vi "SeqEditor_StepOpen.vi"(8 "error in (no error)":errorcluster, 11 "NLTest in":refnum<class "NLTest.lvclass">) -> (0 "error out":errorcluster, 3 "NLTest out":refnum<class "NLTest.lvclass">)   [LabVIEW 2017, in "NLTest.lvclass"]
uses:
  NLTest.lvclass
  NLTest.lvclass/NLTest.ctl
  VISTEP.ctl
  VISTEP_class_INOUTPUT.ctl
  VISTEP_class_INOUTPUT_TYPE.ctl
  VISTEP_class_steptestclass.ctl
panel:
  # "某个步骤被打开，加载PARAM MLST"
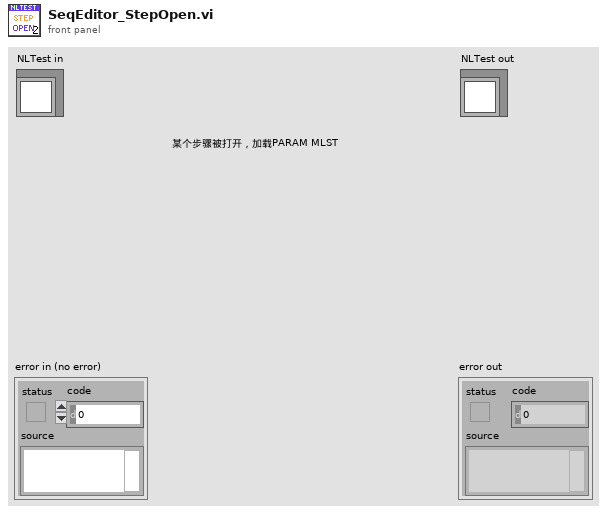
[diagram p1: front panel]
types:
  T1 = typedef "NLTest.lvclass/VISTEP.ctl" = cluster{"My":cluster{"VIpath":T2, "VIname":T2, "Loop":T2, "Skip":T2, "FailStop":T2, "StepClass":T2, "StringTest-Source":T2, "StringTest-Lim":T2, "BoolTest-Source":T2, "BoolTest-Lim":T2, "NumberTest-OP":T2, "NumberTest-Source":T2, "NumberTest-LimA":T2, "NumberTest-LimB":T2}, "INPUT":T2[], "OUTPUT":T2[]}
  T2 = typedef "NLTest.lvclass/VISTEP_class_INOUTPUT.ctl" = cluster{"ITEM":string, "DATA":string, "TYPE":T3, "TYPEDATA":string, "SV":bool, "clusterchain":refnum<vi>[]}
  T3 = typedef "NLTest.lvclass/VISTEP_class_INOUTPUT_TYPE.ctl" = enum16{"Number", "String", "Bool", "Enum", "Path", "VISA", "NA"}
  T4 = typedef "NLTest.lvclass/VISTEP_class_steptestclass.ctl" = enum16{"NotaTest", "StringTest", "BoolTest", "NumberTest", "NULL"}
  T5 = cluster{"ITEM":string, "TYPE":T3, "TYPEDATA":string}
  T6 = cluster{"VIpath":T2, "VIname":T2, "Loop":T2, "Skip":T2, "FailStop":T2, "StepClass":T2, "StringTest-Source":T2, "StringTest-Lim":T2, "BoolTest-Source":T2, "BoolTest-Lim":T2, "NumberTest-OP":T2, "NumberTest-Source":T2, "NumberTest-LimA":T2, "NumberTest-LimB":T2}
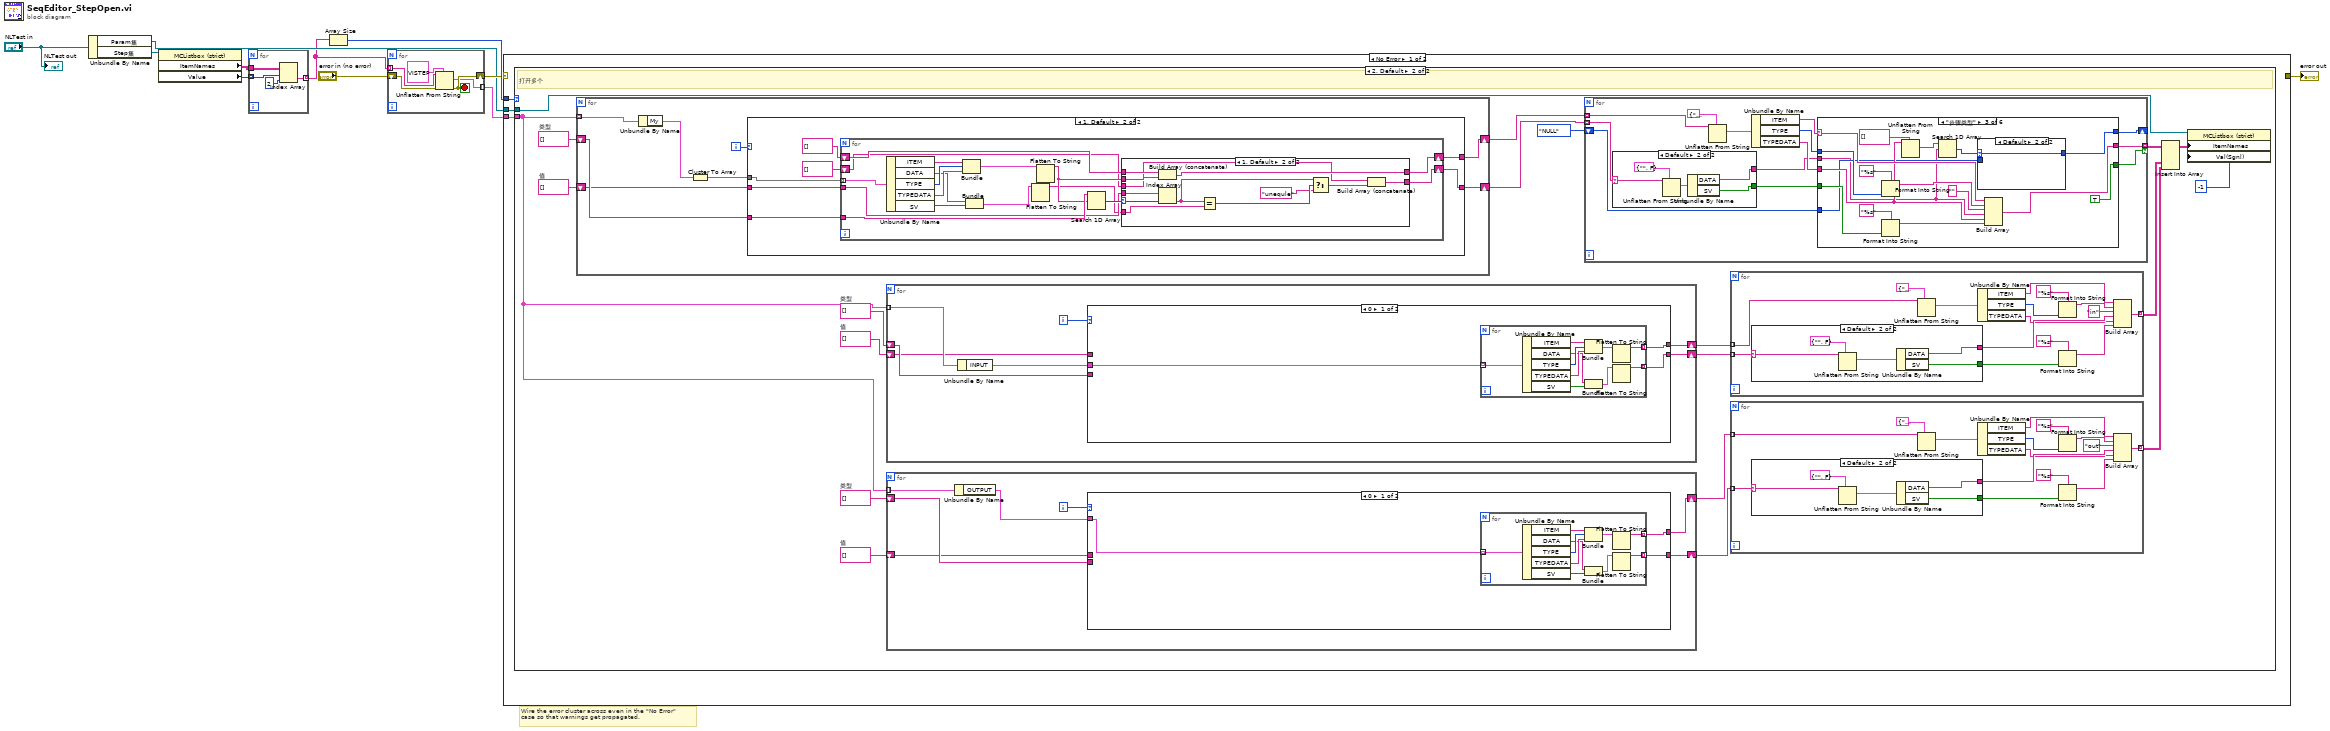
[diagram p0: block diagram]
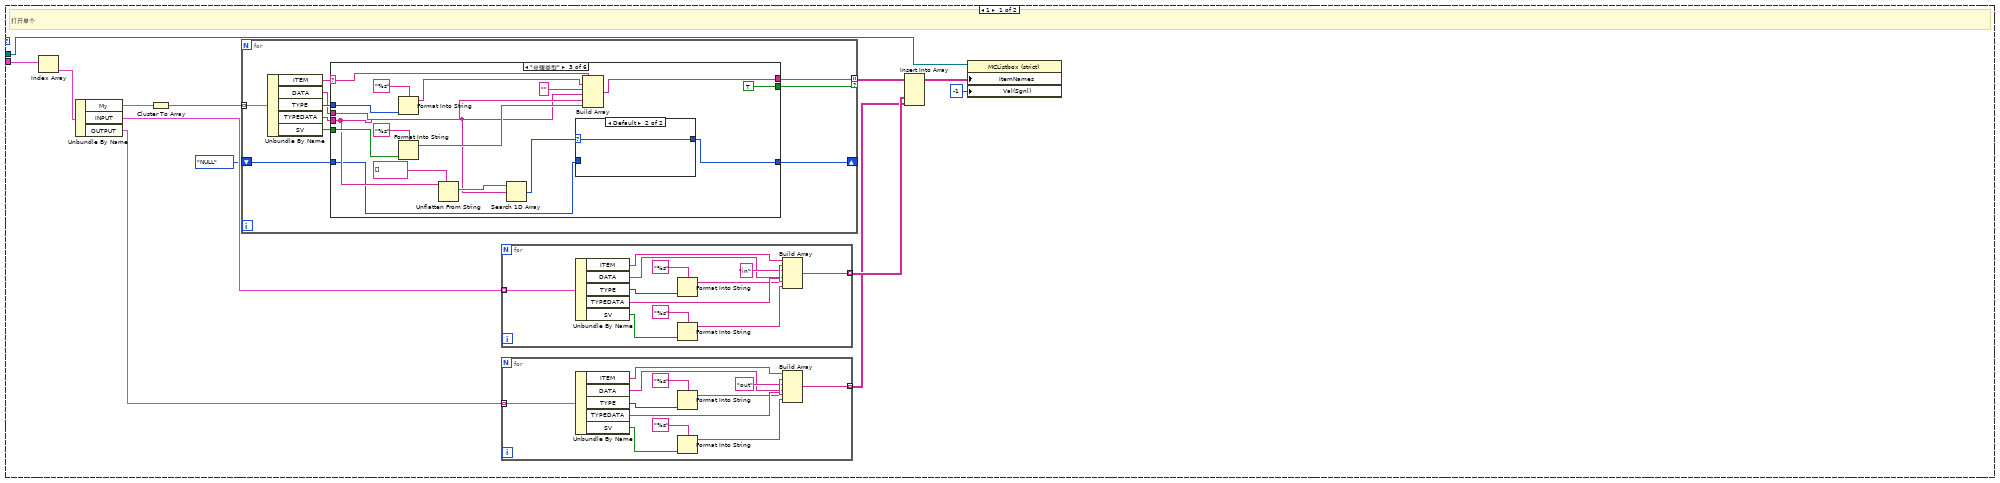
[diagram p2: hidden frame]
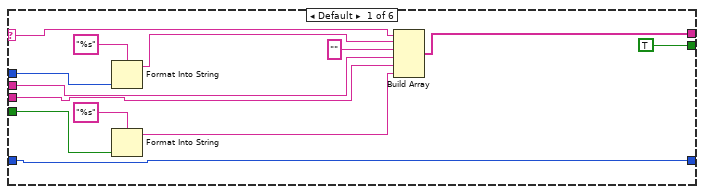
[diagram p3: hidden frame]
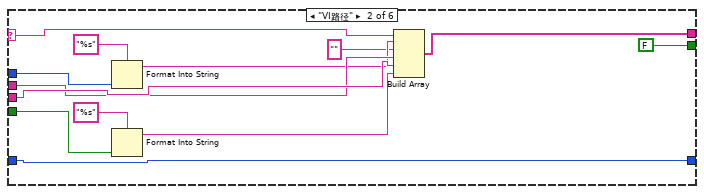
[diagram p4: hidden frame]
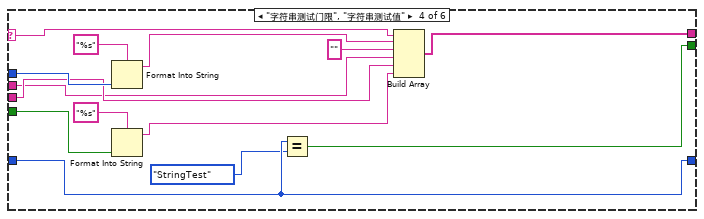
[diagram p6: hidden frame]
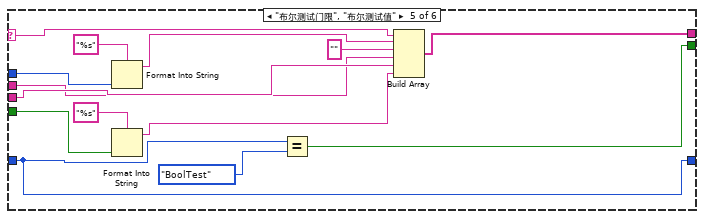
[diagram p7: hidden frame]
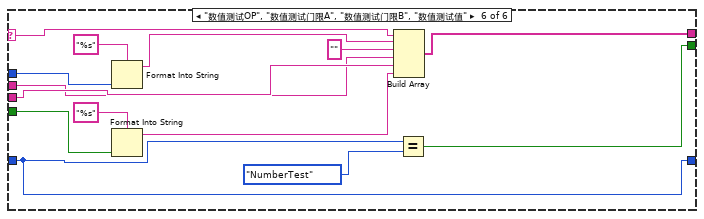
[diagram p8: hidden frame]
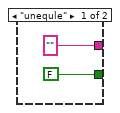
[diagram p9: hidden frame]
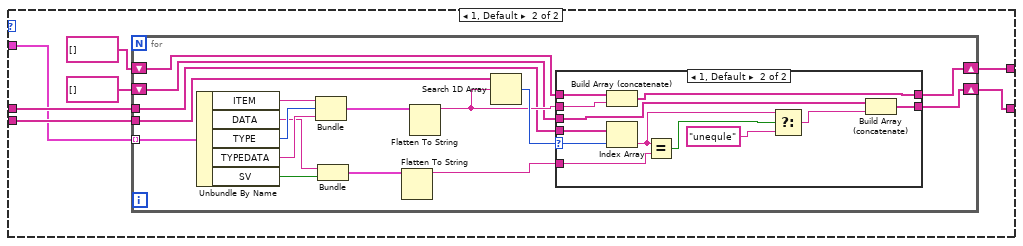
[diagram p10: hidden frame]
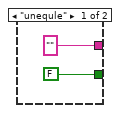
[diagram p12: hidden frame]
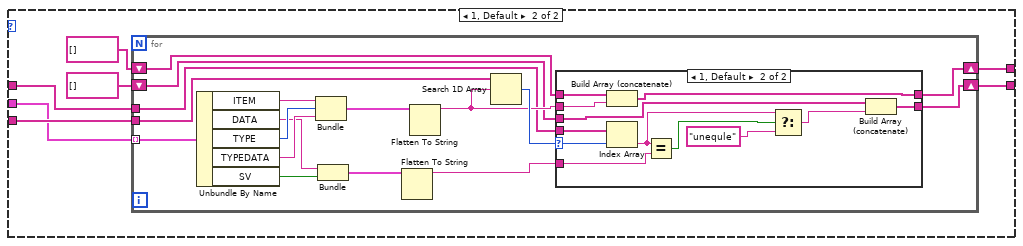
[diagram p13: hidden frame]
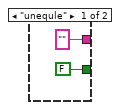
[diagram p15: hidden frame]
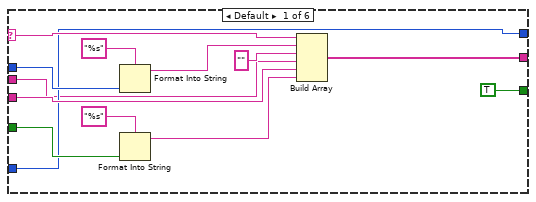
[diagram p16: hidden frame]
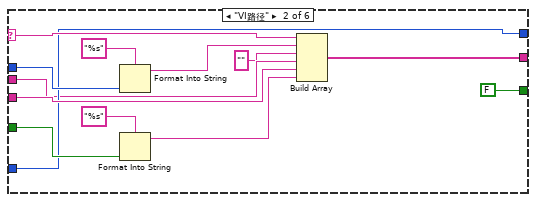
[diagram p17: hidden frame]
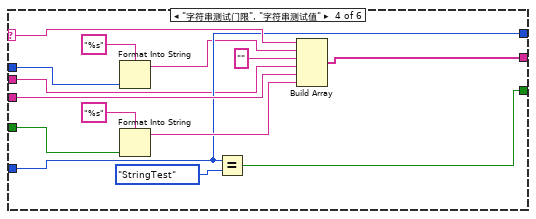
[diagram p19: hidden frame]
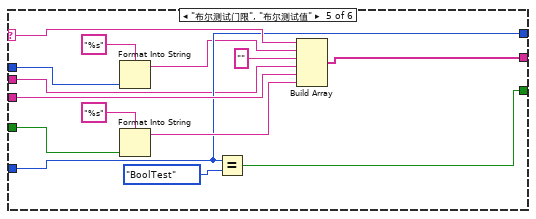
[diagram p20: hidden frame]
diagram:
  # "Wire the error cluster across even in the \"No Error\"\ncase so that warnings get propagated."
  n1 = Unbundle By Name("NLTest in") -> ("Param集"=w5:refnum<vi>, "Step集"=w3:refnum<vi>)
  n2 = property class="MCListbox (strict)"(reference=w3) -> ("ItemNames"=w4:string[][], "Value"=w2:i32[])  [unwired: 1 in, 2 out]
  n3 = for {
    tunnel: w4 -> [w15]
    tunnel: w2 -> [w14] mode=indexing
    tunnel: [w12] -> w1 mode=indexing
    n4 = Index Array(array=w15, index (row)=w14, index (col)=2 ("disabled index (col)")) -> (element=w12:string)
  }
  n5 = Array Size(array=w1) -> (size(s)=w10:i32)
  n6 = for {
    tunnel: w1 -> [w19] mode=indexing
    shift-right: [w17] -> w9
    shift-left: "error in (no error)" -> [w18]
    tunnel: [w16] -> w7 mode=indexing
    stop <- w17 stop-if-true
    n7 = Unflatten From String(type=T1 {"My"={"VIpath"={"ITEM"="VI路径", "DATA"="", "TYPE"=enum."Path", "TYPEDATA"="", "SV"=FALSE, "clusterchain"=[]}, "VIname"={"ITEM"="步骤名称", "DATA"="", "TYPE"=enum."String", "TYPEDATA"="", "SV"=FALSE, "clusterchain"=[]}, "Loop"={"ITEM"="重测次数", "DATA"="1", "TYPE"=enum."Number", "TYPEDATA"="", "SV"=FALSE, "clusterchain"=[]}, "Skip"={"ITEM"="跳过步骤", "DATA"="FALSE", "TYPE"=enum."Bool", "TYPEDATA"="", "SV"=FALSE, "clusterchain"=[]}, "FailStop"={"ITEM"="失败停止", "DATA"="FALSE", "TYPE"=enum."Bool", "TYPEDATA"="", "SV"=FALSE, "clusterchain"=[]}, "StepClass"={"ITEM"="步骤类型", "DATA"="NotaTEST", "TYPE"=enum."Enum", "TYPEDATA"="", "SV"=FALSE, "clusterchain"=[]}, "StringTest-Source"={"ITEM"="字符串测试值", "DATA"="", "TYPE"=enum."String", "TYPEDATA"="", "SV"=FALSE, "clusterchain"=[]}, "StringTest-Lim"={"ITEM"="字符串测试门限", "DATA"="", "TYPE"=enum."String", "TYPEDATA"="", "SV"=FALSE, "clusterchain"=[]}, "BoolTest-Source"={"ITEM"="布尔测试值", "DATA"="", "TYPE"=enum."Bool", "TYPEDATA"="", "SV"=FALSE, "clusterchain"=[]}, "BoolTest-Lim"={"ITEM"="布尔测试门限", "DATA"="", "TYPE"=enum."Bool", "TYPEDATA"="", "SV"=FALSE, "clusterchain"=[]}, "NumberTest-OP"={"ITEM"="数值测试OP", "DATA"="", "TYPE"=enum."Enum", "TYPEDATA"="", "SV"=FALSE, "clusterchain"=[]}, "NumberTest-Source"={"ITEM"="数值测试值", "DATA"="", "TYPE"=enum."Number", "TYPEDATA"="", "SV"=FALSE, "clusterchain"=[]}, "NumberTest-LimA"={"ITEM"="数值测试门限A", "DATA"="", "TYPE"=enum."Number", "TYPEDATA"="", "SV"=FALSE, "clusterchain"=[]}, "NumberTest-LimB"={"ITEM"="数值测试门限B", "DATA"="", "TYPE"=enum."Number", "TYPEDATA"="", "SV"=FALSE, "clusterchain"=[]}}, "INPUT"=[], "OUTPUT"=[]} ("步骤结构"), binary string=w19, error in (no error)=w18) -> (value=w16:T1, error out=w17:errorcluster)  [unwired: 2 in, 1 out]
  }
  n8 = case shown="No Error" w9 {
    selector: w9 -> [_ w504]
    tunnel: w10 -> [w23 _]
    tunnel: [_ w504] -> w8
    tunnel: w7 -> [w22 _]
    tunnel: w5 -> [w21 _]
    frame No Error {
      n9 = case shown="2, Default" w23 {
        tunnel: w22 -> [w36 w160]
        tunnel: w21 -> [w32 w177]
        frame 1 {
          # "打开单个"
          n10 = Index Array(array=w36) -> (element=w35:T1)  [unwired: 1 in]
          n11 = Unbundle By Name(w35) -> ("My"=w28:T6, "INPUT"=w34:T2[], "OUTPUT"=w33:T2[])
          n12 = Cluster To Array(cluster=w28) -> (array=w25:T2[])
          n13 = for {
            tunnel: w25 -> [w46] mode=indexing
            tunnel: [w41] -> w27 mode=indexing if=w37
            shift-right: [w39] -> _
            shift-left: VISTEP_class_steptestclass."NULL" ("步骤类型") -> [w38]
            n14 = Unbundle By Name(w46) -> ("ITEM"=w40:string, "DATA"=w43:string, "TYPE"=w45:T3, "TYPEDATA"=w42:string, "SV"=w44:bool)
            n15 = case shown="\"步骤类型\"" w40 {
              selector: w40 -> [w52 w65 w83 w98 w112 w126]
              tunnel: w45 -> [w59 w72 w89 w105 w119 w133]
              tunnel: w44 -> [w58 w71 w88 w104 w118 w132]
              tunnel: w43 -> [w47 w62 w73 w92 w106 w120]
              tunnel: w42 -> [w57 w70 w82 w103 w117 w131]
              tunnel: [w56 w69 w87 w102 w116 w130] -> w41
              tunnel: [w51 w64 w78 w97 w111 w125] -> w39
              tunnel: w38 -> [w51 w64 w77 w97 w111 w125]
              tunnel: [TRUE FALSE TRUE w95 w109 w123] -> w37
              frame Default {
                n16 = Format Into String(format string="%s", w59) -> (resulting string=w49:string)  [unwired: 2 in, 1 out]
                n17 = Format Into String(format string="%s", w58) -> (resulting string=w53:string)  [unwired: 2 in, 1 out]
                n18 = Build Array(w52, w49, "" ("element"), w47, w57, w53) -> (w56:string[])
              }
              frame "VI路径" {
                n19 = Format Into String(format string="%s", w72) -> (resulting string=w61:string)  [unwired: 2 in, 1 out]
                n20 = Format Into String(format string="%s", w71) -> (resulting string=w66:string)  [unwired: 2 in, 1 out]
                n21 = Build Array(w65, w61, "" ("element"), w62, w70, w66) -> (w69:string[])
              }
              frame "步骤类型" {
                n22 = Format Into String(format string="%s", w89) -> (resulting string=w75:string)  [unwired: 2 in, 1 out]
                n23 = Format Into String(format string="%s", w88) -> (resulting string=w84:string)  [unwired: 2 in, 1 out]
                n24 = Unflatten From String(type=string[] [], binary string=w82) -> (value=w80:string[])  [unwired: 3 in, 2 out]
                n25 = Search 1D Array(1D array=w80, element=w73) -> (index of element=w79:i32)  [unwired: 1 in]
                n26 = case shown="Default" w79 {
                  selector: w79 -> [_ w91]
                  tunnel: [w90 w91] -> w78
                  tunnel: w77 -> [w90 _]
                  frame -1 {
                  }
                  frame Default {
                  }
                }
                n27 = Build Array(w83, w75, "" ("element"), w73, w82, w84) -> (w87:string[])
              }
              frame "字符串测试门限", "字符串测试值" {
                n28 = Format Into String(format string="%s", w105) -> (resulting string=w94:string)  [unwired: 2 in, 1 out]
                n29 = Format Into String(format string="%s", w104) -> (resulting string=w99:string)  [unwired: 2 in, 1 out]
                n30 = Equal?(x=w97, y=VISTEP_class_steptestclass."StringTest" ("步骤类型")) -> (x = y?=w95:bool)
                n31 = Build Array(w98, w94, "" ("element"), w92, w103, w99) -> (w102:string[])
              }
              frame "布尔测试门限", "布尔测试值" {
                n32 = Format Into String(format string="%s", w119) -> (resulting string=w108:string)  [unwired: 2 in, 1 out]
                n33 = Format Into String(format string="%s", w118) -> (resulting string=w113:string)  [unwired: 2 in, 1 out]
                n34 = Equal?(x=w111, y=VISTEP_class_steptestclass."BoolTest" ("步骤类型")) -> (x = y?=w109:bool)
                n35 = Build Array(w112, w108, "" ("element"), w106, w117, w113) -> (w116:string[])
              }
              frame "数值测试OP", "数值测试门限A", "数值测试门限B", "数值测试值" {
                n36 = Format Into String(format string="%s", w133) -> (resulting string=w122:string)  [unwired: 2 in, 1 out]
                n37 = Format Into String(format string="%s", w132) -> (resulting string=w127:string)  [unwired: 2 in, 1 out]
                n38 = Build Array(w126, w122, "" ("element"), w120, w131, w127) -> (w130:string[])
                n39 = Equal?(x=w125, y=VISTEP_class_steptestclass."NumberTest" ("步骤类型")) -> (x = y?=w123:bool)
              }
            }
          }
          n40 = for {
            tunnel: w34 -> [w157] mode=indexing
            tunnel: [w150] -> w31 mode=indexing
            n41 = Unbundle By Name(w157) -> ("ITEM"=w149:string, "DATA"=w146:string, "TYPE"=w156:T3, "TYPEDATA"=w152:string, "SV"=w153:bool)
            n42 = Format Into String(format string="%s", w156) -> (resulting string=w148:string)  [unwired: 2 in, 1 out]
            n43 = Format Into String(format string="%s", w153) -> (resulting string=w151:string)  [unwired: 2 in, 1 out]
            n44 = Build Array(w149, w148, "in" ("element"), w146, w152, w151) -> (w150:string[])
          }
          n45 = for {
            tunnel: w33 -> [w145] mode=indexing
            tunnel: [w138] -> w30 mode=indexing
            n46 = Unbundle By Name(w145) -> ("ITEM"=w137:string, "DATA"=w134:string, "TYPE"=w144:T3, "TYPEDATA"=w140:string, "SV"=w141:bool)
            n47 = Format Into String(format string="%s", w144) -> (resulting string=w136:string)  [unwired: 2 in, 1 out]
            n48 = Format Into String(format string="%s", w141) -> (resulting string=w139:string)  [unwired: 2 in, 1 out]
            n49 = Build Array(w137, w136, "out" ("element"), w134, w140, w139) -> (w138:string[])
          }
          n50 = Insert Into Array(array=w27, new element #1=w31, new element #2=w30) -> (w29:string[][])  [unwired: 2 in]
          n51 = property class="MCListbox (strict)"(reference=w32, "ItemNames"=w29, "Val(Sgnl)"=-1 ("Value (Signaling)")) -> ()  [unwired: 1 in, 2 out]
        }
        frame 2, Default {
          w162 = string[] []  # 值
          w161 = string[] []  # 类型
          w168 = string[] []  # 值
          w169 = string[] []  # 类型
          w175 = string[] []  # 值
          w176 = string[] []  # 类型
          # "打开多个"
          n52 = for {
            tunnel: w160 -> [w451] mode=indexing
            shift-right: [w448] -> w173
            shift-left: w176 -> [w447]
            shift-right: [w446] -> w172
            shift-left: w175 -> [w445]
            i -> [w450]
            n53 = Unbundle By Name(w451) -> ("My"=w452:T6)
            n54 = Cluster To Array(cluster=w452) -> (array=w449:T2[])
            n55 = case shown="1, Default" w450 {
              tunnel: w449 -> [w455 w472]
              tunnel: [w454 w469] -> w448
              tunnel: w447 -> [_ w471]
              tunnel: [w453 w466] -> w446
              tunnel: w445 -> [_ w467]
              frame 0 {
                n56 = for {
                  tunnel: w455 -> [w465] mode=indexing
                  tunnel: [w460] -> w454 mode=indexing
                  tunnel: [w456] -> w453 mode=indexing
                  n57 = Unbundle By Name(w465) -> ("ITEM"=w464:string, "DATA"=w459:string, "TYPE"=w463:T3, "TYPEDATA"=w462:string, "SV"=w458:bool)
                  n58 = Bundle("ITEM"=w464, "TYPE"=w463, "TYPEDATA"=w462) -> (w461:T5)  [unwired: 1 in]
                  n59 = Bundle("DATA"=w459, "SV"=w458) -> (w457:cluster{"DATA":string, "SV":bool})  [unwired: 1 in]
                  n60 = Flatten To String(anything=w461) -> (data string=w460:string)  [unwired: 3 in, 2 out]
                  n61 = Flatten To String(anything=w457) -> (data string=w456:string)  [unwired: 3 in, 2 out]
                }
              }
              frame 1, Default {
                n62 = for {
                  tunnel: w472 -> [w489] mode=indexing
                  shift-right: [w482] -> w469
                  shift-left: string[] [] -> [w481]
                  tunnel: w471 -> [w484]
                  shift-right: [w476] -> w466
                  shift-left: string[] [] -> [w475]
                  tunnel: w467 -> [w474]
                  n63 = Unbundle By Name(w489) -> ("ITEM"=w488:string, "DATA"=w478:string, "TYPE"=w487:T3, "TYPEDATA"=w486:string, "SV"=w477:bool)
                  n64 = Bundle("ITEM"=w488, "TYPE"=w487, "TYPEDATA"=w486) -> (w485:T5)  [unwired: 1 in]
                  n65 = Bundle("DATA"=w478, "SV"=w477) -> (w479:cluster{"DATA":string, "SV":bool})  [unwired: 1 in]
                  n66 = Flatten To String(anything=w479) -> (data string=w473:string)  [unwired: 3 in, 2 out]
                  n67 = Flatten To String(anything=w485) -> (data string=w480:string)  [unwired: 3 in, 2 out]
                  n68 = Search 1D Array(1D array=w484, element=w480) -> (index of element=w483:i32)  [unwired: 1 in]
                  n69 = case shown="1, Default" w483 {
                    selector: w483 -> [_ w492]
                    tunnel: [w491 w502] -> w482
                    tunnel: w481 -> [w491 w503]
                    tunnel: w480 -> [_ w501]
                    tunnel: [w490 w494] -> w476
                    tunnel: w475 -> [w490 w496]
                    tunnel: w474 -> [_ w500]
                    tunnel: w473 -> [_ w499]
                    frame -1 {
                    }
                    frame 1, Default {
                      n70 = Build Array (concatenate)(w503, w501) -> (w502:string[])
                      n71 = Index Array(array=w500, index=w492) -> (element=w497:string)
                      n72 = Equal?(x=w497, y=w499) -> (x = y?=w498:bool)
                      n73 = Select(t=w497, s=w498, f="unequle") -> (s? t:f=w495:string)
                      n74 = Build Array (concatenate)(w496, w495) -> (w494:string[])
                    }
                  }
                }
              }
            }
          }
          n75 = for {
            tunnel: w160 -> [w286] mode=indexing
            shift-right: [w283] -> w167
            shift-left: w169 -> [w282]
            shift-right: [w281] -> w166
            shift-left: w168 -> [w280]
            i -> [w285]
            n76 = Unbundle By Name(w286) -> ("INPUT"=w284:T2[])
            n77 = case shown="0" w285 {
              tunnel: w284 -> [w287 w300]
              tunnel: [w289 w304] -> w283
              tunnel: w282 -> [_ w306]
              tunnel: [w288 w301] -> w281
              tunnel: w280 -> [_ w302]
              frame 0 {
                n78 = for {
                  tunnel: w287 -> [w299] mode=indexing
                  tunnel: [w294] -> w289 mode=indexing
                  tunnel: [w290] -> w288 mode=indexing
                  n79 = Unbundle By Name(w299) -> ("ITEM"=w298:string, "DATA"=w293:string, "TYPE"=w297:T3, "TYPEDATA"=w296:string, "SV"=w292:bool)
                  n80 = Bundle("ITEM"=w298, "TYPE"=w297, "TYPEDATA"=w296) -> (w295:T5)  [unwired: 1 in]
                  n81 = Bundle("DATA"=w293, "SV"=w292) -> (w291:cluster{"DATA":string, "SV":bool})  [unwired: 1 in]
                  n82 = Flatten To String(anything=w295) -> (data string=w294:string)  [unwired: 3 in, 2 out]
                  n83 = Flatten To String(anything=w291) -> (data string=w290:string)  [unwired: 3 in, 2 out]
                }
              }
              frame 1, Default {
                n84 = for {
                  tunnel: w300 -> [w323] mode=indexing
                  shift-right: [w316] -> w304
                  shift-left: string[] [] -> [w315]
                  tunnel: w306 -> [w318]
                  shift-right: [w310] -> w301
                  shift-left: string[] [] -> [w309]
                  tunnel: w302 -> [w308]
                  n85 = Unbundle By Name(w323) -> ("ITEM"=w322:string, "DATA"=w312:string, "TYPE"=w321:T3, "TYPEDATA"=w320:string, "SV"=w311:bool)
                  n86 = Bundle("ITEM"=w322, "TYPE"=w321, "TYPEDATA"=w320) -> (w319:T5)  [unwired: 1 in]
                  n87 = Bundle("DATA"=w312, "SV"=w311) -> (w313:cluster{"DATA":string, "SV":bool})  [unwired: 1 in]
                  n88 = Flatten To String(anything=w313) -> (data string=w307:string)  [unwired: 3 in, 2 out]
                  n89 = Flatten To String(anything=w319) -> (data string=w314:string)  [unwired: 3 in, 2 out]
                  n90 = Search 1D Array(1D array=w318, element=w314) -> (index of element=w317:i32)  [unwired: 1 in]
                  n91 = case shown="1, Default" w317 {
                    selector: w317 -> [_ w326]
                    tunnel: [w325 w336] -> w316
                    tunnel: w315 -> [w325 w337]
                    tunnel: w314 -> [_ w335]
                    tunnel: [w324 w328] -> w310
                    tunnel: w309 -> [w324 w330]
                    tunnel: w308 -> [_ w334]
                    tunnel: w307 -> [_ w333]
                    frame -1 {
                    }
                    frame 1, Default {
                      n92 = Build Array (concatenate)(w337, w335) -> (w336:string[])
                      n93 = Index Array(array=w334, index=w326) -> (element=w331:string)
                      n94 = Equal?(x=w331, y=w333) -> (x = y?=w332:bool)
                      n95 = Select(t=w331, s=w332, f="unequle") -> (s? t:f=w329:string)
                      n96 = Build Array (concatenate)(w330, w329) -> (w328:string[])
                    }
                  }
                }
              }
            }
          }
          n97 = for {
            tunnel: w160 -> [w206] mode=indexing
            shift-right: [w203] -> w163
            shift-left: w161 -> [w202]
            shift-right: [w201] -> w164
            shift-left: w162 -> [w200]
            i -> [w205]
            n98 = Unbundle By Name(w206) -> ("OUTPUT"=w204:T2[])
            n99 = case shown="0" w205 {
              tunnel: w204 -> [w207 w220]
              tunnel: [w209 w224] -> w203
              tunnel: w202 -> [_ w226]
              tunnel: [w208 w221] -> w201
              tunnel: w200 -> [_ w222]
              frame 0 {
                n100 = for {
                  tunnel: w207 -> [w219] mode=indexing
                  tunnel: [w214] -> w209 mode=indexing
                  tunnel: [w210] -> w208 mode=indexing
                  n101 = Unbundle By Name(w219) -> ("ITEM"=w218:string, "DATA"=w213:string, "TYPE"=w217:T3, "TYPEDATA"=w216:string, "SV"=w212:bool)
                  n102 = Bundle("ITEM"=w218, "TYPE"=w217, "TYPEDATA"=w216) -> (w215:T5)  [unwired: 1 in]
                  n103 = Bundle("DATA"=w213, "SV"=w212) -> (w211:cluster{"DATA":string, "SV":bool})  [unwired: 1 in]
                  n104 = Flatten To String(anything=w215) -> (data string=w214:string)  [unwired: 3 in, 2 out]
                  n105 = Flatten To String(anything=w211) -> (data string=w210:string)  [unwired: 3 in, 2 out]
                }
              }
              frame 1, Default {
                n106 = for {
                  tunnel: w220 -> [w243] mode=indexing
                  shift-right: [w236] -> w224
                  shift-left: string[] [] -> [w235]
                  tunnel: w226 -> [w238]
                  shift-right: [w230] -> w221
                  shift-left: string[] [] -> [w229]
                  tunnel: w222 -> [w228]
                  n107 = Unbundle By Name(w243) -> ("ITEM"=w242:string, "DATA"=w232:string, "TYPE"=w241:T3, "TYPEDATA"=w240:string, "SV"=w231:bool)
                  n108 = Bundle("ITEM"=w242, "TYPE"=w241, "TYPEDATA"=w240) -> (w239:T5)  [unwired: 1 in]
                  n109 = Bundle("DATA"=w232, "SV"=w231) -> (w233:cluster{"DATA":string, "SV":bool})  [unwired: 1 in]
                  n110 = Flatten To String(anything=w233) -> (data string=w227:string)  [unwired: 3 in, 2 out]
                  n111 = Flatten To String(anything=w239) -> (data string=w234:string)  [unwired: 3 in, 2 out]
                  n112 = Search 1D Array(1D array=w238, element=w234) -> (index of element=w237:i32)  [unwired: 1 in]
                  n113 = case shown="1, Default" w237 {
                    selector: w237 -> [_ w246]
                    tunnel: [w245 w256] -> w236
                    tunnel: w235 -> [w245 w257]
                    tunnel: w234 -> [_ w255]
                    tunnel: [w244 w248] -> w230
                    tunnel: w229 -> [w244 w250]
                    tunnel: w228 -> [_ w254]
                    tunnel: w227 -> [_ w253]
                    frame -1 {
                    }
                    frame 1, Default {
                      n114 = Build Array (concatenate)(w257, w255) -> (w256:string[])
                      n115 = Index Array(array=w254, index=w246) -> (element=w251:string)
                      n116 = Equal?(x=w251, y=w253) -> (x = y?=w252:bool)
                      n117 = Select(t=w251, s=w252, f="unequle") -> (s? t:f=w249:string)
                      n118 = Build Array (concatenate)(w250, w249) -> (w248:string[])
                    }
                  }
                }
              }
            }
          }
          n119 = for {
            tunnel: [w350] -> w171 mode=indexing if=w347
            shift-right: [w349] -> _
            shift-left: VISTEP_class_steptestclass."NULL" ("步骤类型") -> [w348]
            tunnel: w173 -> [w345] mode=indexing
            tunnel: w172 -> [w340] mode=indexing
            n120 = case shown="Default" w340 {
              selector: w340 -> [_ w356]
              tunnel: ["" w354] -> w339
              tunnel: [FALSE w353] -> w338
              frame "unequle" {
              }
              frame Default {
                n121 = Unflatten From String(type=cluster{"DATA":string, "SV":bool} {"DATA"="", "SV"=FALSE} ("output cluster"), binary string=w356) -> (value=w355:cluster{"DATA":string, "SV":bool})  [unwired: 3 in, 2 out]
                n122 = Unbundle By Name(w355) -> ("DATA"=w354:string, "SV"=w353:bool)
              }
            }
            n123 = Unflatten From String(type=T5 {"ITEM"="", "TYPE"=enum."Number", "TYPEDATA"=""} ("output cluster"), binary string=w345) -> (value=w344:T5)  [unwired: 3 in, 2 out]
            n124 = Unbundle By Name(w344) -> ("ITEM"=w343:string, "TYPE"=w342:T3, "TYPEDATA"=w341:string)
            n125 = case shown="\"步骤类型\"" w343 {
              selector: w343 -> [w363 w376 w394 w409 w423 w437]
              tunnel: w342 -> [w370 w383 w400 w416 w430 w444]
              tunnel: w338 -> [w369 w382 w399 w415 w429 w443]
              tunnel: w339 -> [w358 w373 w384 w403 w417 w431]
              tunnel: w341 -> [w368 w381 w393 w414 w428 w442]
              tunnel: [w367 w380 w398 w413 w427 w441] -> w350
              tunnel: [w362 w375 w389 w408 w422 w436] -> w349
              tunnel: w348 -> [w362 w375 w388 w408 w422 w436]
              tunnel: [TRUE FALSE TRUE w406 w420 w434] -> w347
              frame Default {
                n126 = Format Into String(format string="%s", w370) -> (resulting string=w360:string)  [unwired: 2 in, 1 out]
                n127 = Format Into String(format string="%s", w369) -> (resulting string=w364:string)  [unwired: 2 in, 1 out]
                n128 = Build Array(w363, w360, "" ("element"), w358, w368, w364) -> (w367:string[])
              }
              frame "VI路径" {
                n129 = Format Into String(format string="%s", w383) -> (resulting string=w372:string)  [unwired: 2 in, 1 out]
                n130 = Format Into String(format string="%s", w382) -> (resulting string=w377:string)  [unwired: 2 in, 1 out]
                n131 = Build Array(w376, w372, "" ("element"), w373, w381, w377) -> (w380:string[])
              }
              frame "步骤类型" {
                n132 = Format Into String(format string="%s", w400) -> (resulting string=w386:string)  [unwired: 2 in, 1 out]
                n133 = Format Into String(format string="%s", w399) -> (resulting string=w395:string)  [unwired: 2 in, 1 out]
                n134 = Unflatten From String(type=string[] [], binary string=w393) -> (value=w391:string[])  [unwired: 3 in, 2 out]
                n135 = Search 1D Array(1D array=w391, element=w384) -> (index of element=w390:i32)  [unwired: 1 in]
                n136 = case shown="Default" w390 {
                  selector: w390 -> [_ w402]
                  tunnel: [w401 w402] -> w389
                  tunnel: w388 -> [w401 _]
                  frame -1 {
                  }
                  frame Default {
                  }
                }
                n137 = Build Array(w394, w386, "" ("element"), w384, w393, w395) -> (w398:string[])
              }
              frame "字符串测试门限", "字符串测试值" {
                n138 = Format Into String(format string="%s", w416) -> (resulting string=w405:string)  [unwired: 2 in, 1 out]
                n139 = Format Into String(format string="%s", w415) -> (resulting string=w410:string)  [unwired: 2 in, 1 out]
                n140 = Equal?(x=w408, y=VISTEP_class_steptestclass."StringTest" ("步骤类型")) -> (x = y?=w406:bool)
                n141 = Build Array(w409, w405, "" ("element"), w403, w414, w410) -> (w413:string[])
              }
              frame "布尔测试门限", "布尔测试值" {
                n142 = Format Into String(format string="%s", w430) -> (resulting string=w419:string)  [unwired: 2 in, 1 out]
                n143 = Format Into String(format string="%s", w429) -> (resulting string=w424:string)  [unwired: 2 in, 1 out]
                n144 = Equal?(x=w422, y=VISTEP_class_steptestclass."BoolTest" ("步骤类型")) -> (x = y?=w420:bool)
                n145 = Build Array(w423, w419, "" ("element"), w417, w428, w424) -> (w427:string[])
              }
              frame "数值测试OP", "数值测试门限A", "数值测试门限B", "数值测试值" {
                n146 = Format Into String(format string="%s", w444) -> (resulting string=w433:string)  [unwired: 2 in, 1 out]
                n147 = Format Into String(format string="%s", w443) -> (resulting string=w438:string)  [unwired: 2 in, 1 out]
                n148 = Build Array(w437, w433, "" ("element"), w431, w442, w438) -> (w441:string[])
                n149 = Equal?(x=w436, y=VISTEP_class_steptestclass."NumberTest" ("步骤类型")) -> (x = y?=w434:bool)
              }
            }
          }
          n150 = for {
            tunnel: [w269] -> w165 mode=indexing
            tunnel: w167 -> [w265] mode=indexing
            tunnel: w166 -> [w263] mode=indexing
            n151 = case shown="Default" w263 {
              selector: w263 -> [_ w278]
              tunnel: ["" w276] -> w261
              tunnel: [FALSE w275] -> w258
              frame "unequle" {
              }
              frame Default {
                n152 = Unflatten From String(type=cluster{"DATA":string, "SV":bool} {"DATA"="", "SV"=FALSE} ("output cluster"), binary string=w278) -> (value=w277:cluster{"DATA":string, "SV":bool})  [unwired: 3 in, 2 out]
                n153 = Unbundle By Name(w277) -> ("DATA"=w276:string, "SV"=w275:bool)
              }
            }
            n154 = Unflatten From String(type=T5 {"ITEM"="", "TYPE"=enum."Number", "TYPEDATA"=""} ("output cluster"), binary string=w265) -> (value=w266:T5)  [unwired: 3 in, 2 out]
            n155 = Unbundle By Name(w266) -> ("ITEM"=w262:string, "TYPE"=w260:T3, "TYPEDATA"=w259:string)
            n156 = Format Into String(format string="%s", w260) -> (resulting string=w268:string)  [unwired: 2 in, 1 out]
            n157 = Format Into String(format string="%s", w258) -> (resulting string=w270:string)  [unwired: 2 in, 1 out]
            n158 = Build Array(w262, w268, "in" ("element"), w261, w259, w270) -> (w269:string[])
          }
          n159 = for {
            tunnel: [w189] -> w159 mode=indexing
            tunnel: w163 -> [w185] mode=indexing
            tunnel: w164 -> [w183] mode=indexing
            n160 = case shown="Default" w183 {
              selector: w183 -> [_ w198]
              tunnel: ["" w196] -> w181
              tunnel: [FALSE w195] -> w178
              frame "unequle" {
              }
              frame Default {
                n161 = Unflatten From String(type=cluster{"DATA":string, "SV":bool} {"DATA"="", "SV"=FALSE} ("output cluster"), binary string=w198) -> (value=w197:cluster{"DATA":string, "SV":bool})  [unwired: 3 in, 2 out]
                n162 = Unbundle By Name(w197) -> ("DATA"=w196:string, "SV"=w195:bool)
              }
            }
            n163 = Unflatten From String(type=T5 {"ITEM"="", "TYPE"=enum."Number", "TYPEDATA"=""} ("output cluster"), binary string=w185) -> (value=w186:T5)  [unwired: 3 in, 2 out]
            n164 = Unbundle By Name(w186) -> ("ITEM"=w182:string, "TYPE"=w180:T3, "TYPEDATA"=w179:string)
            n165 = Format Into String(format string="%s", w180) -> (resulting string=w188:string)  [unwired: 2 in, 1 out]
            n166 = Format Into String(format string="%s", w178) -> (resulting string=w190:string)  [unwired: 2 in, 1 out]
            n167 = Build Array(w182, w188, "out" ("element"), w181, w179, w190) -> (w189:string[])
          }
          n168 = Insert Into Array(array=w171, new element #1=w165, new element #2=w159) -> (w170:string[][])  [unwired: 2 in]
          n169 = property class="MCListbox (strict)"(reference=w177, "ItemNames"=w170, "Val(Sgnl)"=-1 ("Value (Signaling)")) -> ()  [unwired: 1 in, 2 out]
        }
      }
    }
    frame Error {
    }
  }
  "error out" <- w8
  "NLTest out" <- "NLTest in"
